vi "InitializeProjectWizardItem.vi"(8 "error in (no error)":errorcluster, 9 "wizard argument":string, 10 "wizard":string, 11 "ProjectWizard in":refnum<class "ProjectWizard.lvclass">) -> (0 "error out":errorcluster, 3 "ProjectWizard out":refnum<class "ProjectWizard.lvclass">)   [LabVIEW 2023, in "GettingStartedWindow.lvlib" / "ProjectWizard.lvclass"]
uses:
  <resource>/modes/FRC/Classes/ProjectWizard/ProjectWizard.lvclass
  <resource>/modes/FRC/Classes/ProjectWizard/ProjectWizard.lvclass/ProjectWizard.ctl
  <resource>/modes/FRC/GettingStartedWindow.lvlib
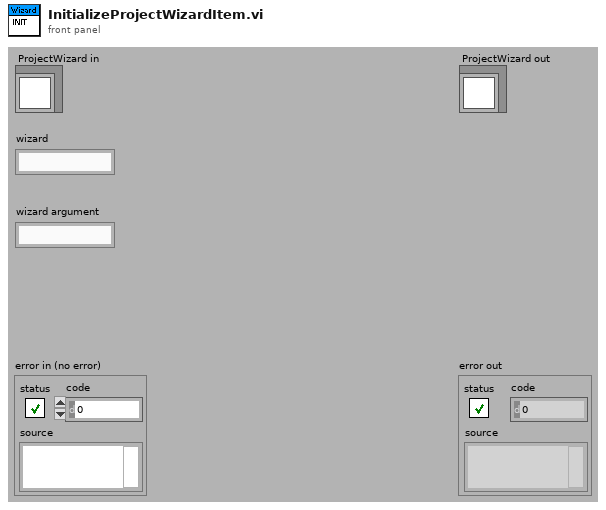
[diagram p1: front panel]
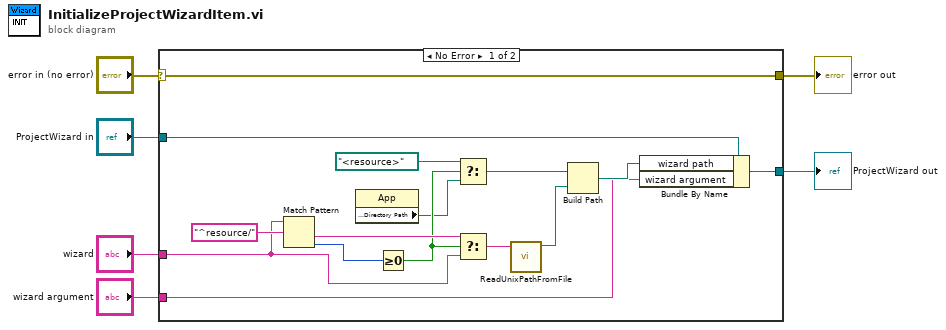
[diagram p0: block diagram]
diagram:
  n1 = case shown="No Error" "error in (no error)" {
    selector: "error in (no error)" -> [w16 w22]
    tunnel: [w16 w22] -> w2
    tunnel: [w17 w23] -> w1
    tunnel: "ProjectWizard in" -> [w18 w23]
    tunnel: "wizard argument" -> [w19 _]
    tunnel: "wizard" -> [w12 _]
    frame No Error {
      n2 = Match Pattern(string=w12, regular expression="^resource/") -> (after substring=w13:string, offset past match=w14:i32)  [unwired: 1 in, 2 out]
      n3 = property class="App"() -> ("Application:Directory Path"=w8:path)  [unwired: 2 in, 2 out]
      n4 = Greater Or Equal To 0?(x=w14) -> (x >= 0?=w10:bool)
      n5 = Select(t=path "<resource>", s=w10, f=w8) -> (s? t:f=w7:path)
      n6 = Select(t=w13, s=w10, f=w12) -> (s? t:f=w11:string)
      n7 = call <resource>:"ReadUnixPathFromFile.vi"("path"=w11) -> ("path"=w21:path)  [unwired: 10 in]
      n8 = Build Path(base path=w7, name or relative path=w21) -> (appended path=w20:path)
      n9 = Bundle By Name(cluster=w18, "wizard path"=w20, "wizard argument"=w19) -> (w17:refnum<class "ProjectWizard.lvclass">)
    }
    frame Error {
    }
  }
  "error out" <- w2
  "ProjectWizard out" <- w1
